vi "Sound_Loop.vi"(0 "Channels":T2, 1 "Sound":bool=TRUE, 5 "Bank":cluster{"Y":dbl[]}[](array[cluster]), 7 "Task ID":u32, 9 "Mixer":T1={"Current"=[], "Position"=0, "Priority"=99, "Music"=FALSE, "MusicPos"=0}, 11 "error in":errorcluster) -> (15 "error out":errorcluster)   [LabVIEW 2020, in "GH_App.lvlib"]
doc: "The sound loop of Main as a subVI, so that it runs in its own execution system (other 2) and never waits for the user interface thread or the picture: Audio_Block until Stop (the sound queue is released at the end of the game)."
uses:
  GH_App.lvlib
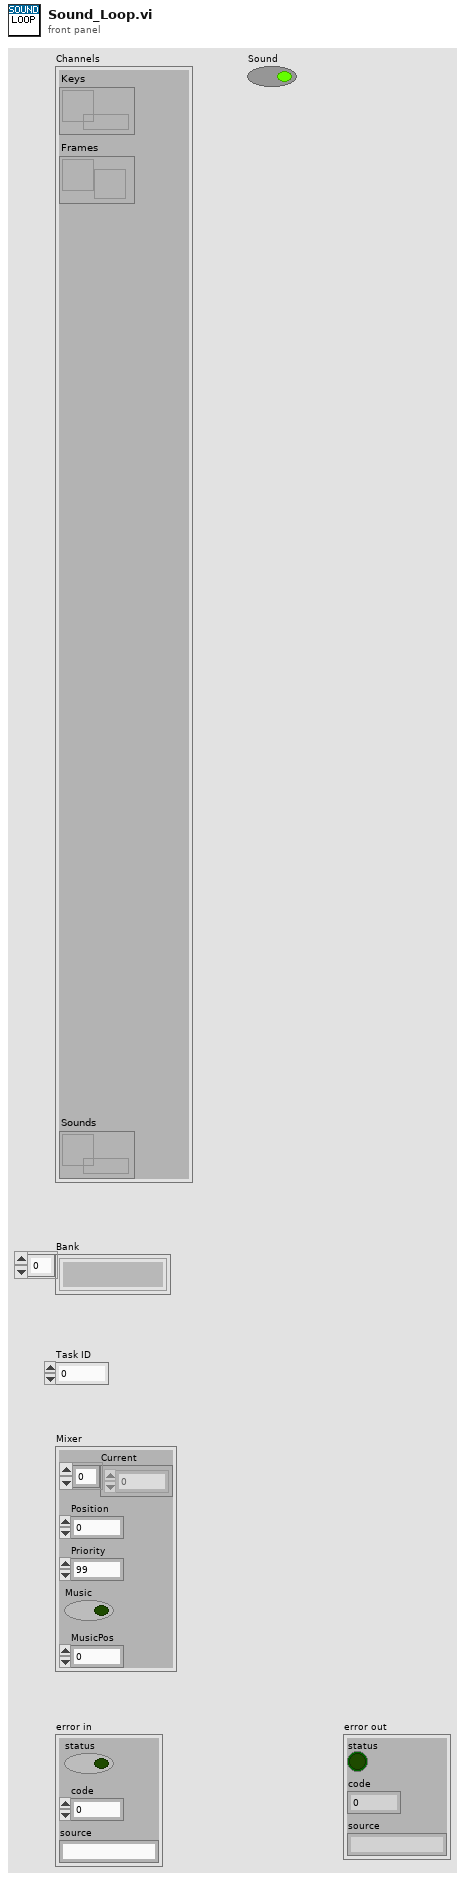
[diagram p1: front panel]
types:
  T1 = cluster{"Current":dbl[], "Position":i32, "Priority":i32, "Music":bool, "MusicPos":i32}
  T2 = cluster{"Keys":refnum<queue>, "Frames":refnum<notifier>, "Sounds":refnum<queue>}
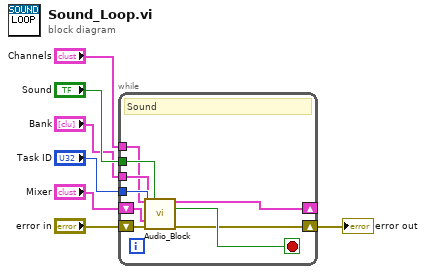
[diagram p0: block diagram]
diagram:
  n1 = while {
    tunnel: "Channels" -> [w8]
    tunnel: "Bank" -> [w9]
    tunnel: "Task ID" -> [w10]
    tunnel: "Sound" -> [w11]
    shift-right: [w13] -> _
    shift-left: "Mixer" -> [w12]
    shift-right: [w15] -> w7
    shift-left: "error in" -> [w14]
    stop <- w16 stop-if-true
    # "Sound"
    n2 = call "Audio_Block.vi"("Channels"=w8, "Sound"=w11, "Bank"=w9, "Task ID"=w10, "Mixer"=w12, "error in"=w14) -> ("Mixer out"=w13:T1, "Stop"=w16:bool, "error out"=w15:errorcluster)  [unwired: 7 in]
  }
  "error out" <- w7
